vi "CloseDevice.vi"(8 "error in (no error)":errorcluster, 11 "id":u16) -> (0 "错误输出":errorcluster)   [LabVIEW 2020]
uses:
  Sprint_Work/SubVI/data/ADIO86.dll
panel:
  out "返回类型":i32
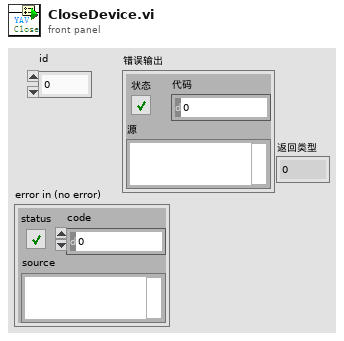
[diagram p1: front panel]
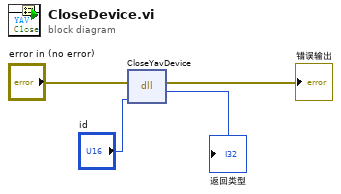
[diagram p0: block diagram]
diagram:
  n1 = dll-call lib="PTH2¡abs CUsers\tæœªæ„ˆä¹…\tDownloads4.è™šæ‹Ÿä»ªå™¨å®žè·µoutputsgithub_prepare_20261104_113201labview-fall-detectionSprint_WorkSubVIdata\nADIO86.dll" fn="CloseYavDevice"(error in="error in (no error)", "ID"="id") -> (error out=→"错误输出":errorcluster, "返回类型"=→"返回类型":i32)  [unwired: 3 in, 1 out]
